vi "Build CE Deploy - Update Project Links.vi"(8 "error in":errorcluster, 10 "Project file":path) -> (0 "error out":errorcluster, 2 "dup Project file":path)   [LabVIEW 2021]
doc: "::: CalcExpress Toolkit :::\nCopyright (c) 2000-2026 Konstantin Shifershteyn. All rights reserved."
panel:
  # "CalcExpress Toolkit\nCopyright (c) 2000-2026 Konstantin Shifershteyn"
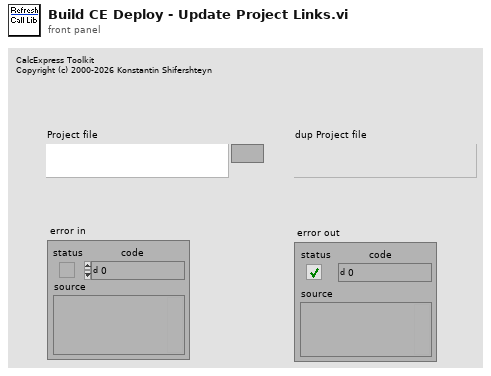
[diagram p1: front panel]
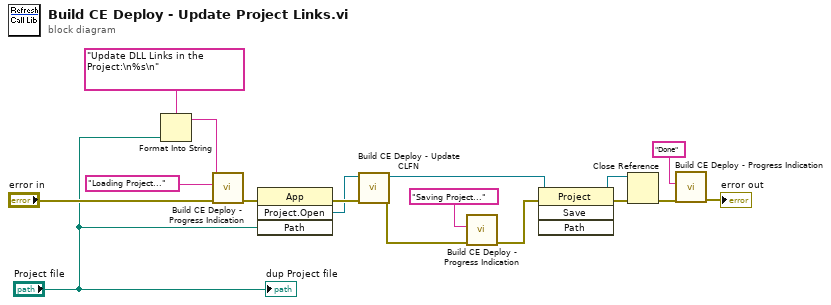
[diagram p0: block diagram]
diagram:
  n1 = Format Into String(format string="Update DLL Links in the Project:\n%s\n", "Project file") -> (resulting string=w10:string)  [unwired: 2 in, 1 out]
  n2 = call "Build CE Deploy - Progress Indication.vi"("error in"="error in", "message 2"="Loading Project...", "message 1"=w10) -> ("error out"=w11:errorcluster)  [unwired: 8 in]
  n3 = invoke class="App" method="Project.Open"(error in=w11, "Path"="Project file") -> (error out=w17:errorcluster, "Project:Open"=w16:refnum<vi>)  [unwired: 2 in, 2 out]
  n4 = call "Build CE Deploy - Update CLFN.vi"("error in"=w17, "Project"=w16) -> ("error out"=w4:errorcluster, "dup Project"=w13:refnum<vi>)  [unwired: 8 in]
  n5 = call "Build CE Deploy - Progress Indication.vi"("error in"=w4, "message 2"="Saving Project...") -> ("error out"=w3:errorcluster)  [unwired: 9 in]
  n6 = invoke class="Project" method="Save"(reference=w13, error in=w3) -> (reference out=w14:refnum<vi>, error out=w15:errorcluster)  [unwired: 2 in, 2 out]
  n7 = Close Reference(reference=w14, error in (no error)=w15) -> (error out=w7:errorcluster)
  n8 = call "Build CE Deploy - Progress Indication.vi"("error in"=w7, "message 2"="Done") -> ("error out"=→"error out":errorcluster)  [unwired: 9 in]
  "dup Project file" <- "Project file"
